vi "Title_Blit.vi"(0 "Title":T2, 5 "Sprites":cluster{"Pix":u8[][], "Mask":u8[][]}[](array[cluster]), 7 "State":T1={"Tick"=0, "Phase"=0, "PhaseTicks"=0, "Level"=1, "Room"=0, "X10"=0, "Y10"=0, "VY10"=0, "Mode"=0, "Facing"=0, "Run"=0, "Vert"=0, "StandY"=0, "EntryX10"=0, "EntryY10"=0, "EntryMode"=0, "Lives"=4, "Score"=0, "NextLife"=10000, "KeyR"=0, "KeyB"=0, "KeyY"=0, "Torch"=FALSE, "FloorPhase"=0, "Dead"=FALSE, "LevelStart"=FALSE, "Quit"=FALSE, "Sound"=0, "Seed"=12345, "DemoStep"=0, "Tiles"=[], "World"=[], "Enemies"=[], "Highscores"=[], "Name"=[0, 0, 0], "Cursor"=0}, 11 "error in":errorcluster) -> (4 "Picture":u8[][](array[numeric]), 15 "error out":errorcluster)   [LabVIEW 2020, in "GH_Render.lvlib"]
doc: "The title screen as one raster (rows x width*3 RGB): title.png holds two pages one below the other - the title image and below it the short help (shown TITLE_HELP ticks after the title card) - with the overlay of the phase on top."
uses:
  GH_Render.lvlib
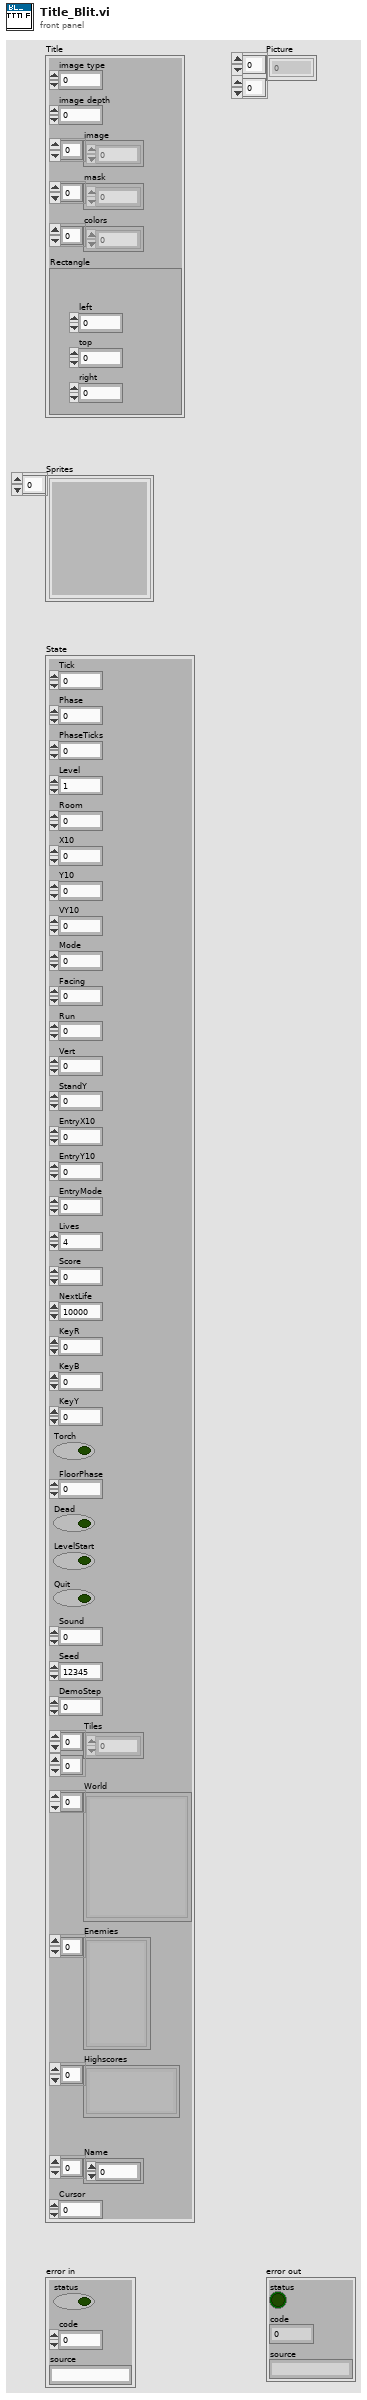
[diagram p1: front panel]
types:
  T1 = cluster{"Tick":u32, "Phase":i32, "PhaseTicks":i32, "Level":i32, "Room":i32, "X10":i32, "Y10":i32, "VY10":i32, "Mode":i32, "Facing":i32, "Run":i32, "Vert":i32, "StandY":i32, "EntryX10":i32, "EntryY10":i32, "EntryMode":i32, "Lives":i32, "Score":i32, "NextLife":i32, "KeyR":i32, "KeyB":i32, "KeyY":i32, "Torch":bool, "FloorPhase":i32, "Dead":bool, "LevelStart":bool, "Quit":bool, "Sound":i32, "Seed":u32, "DemoStep":i32, "Tiles":u8[][], "World":cluster{"ID":string, "Depth":i32, "Column":i32, "Tiles":u8[][]}[], "Enemies":cluster{"Kind":i32, "X10":i32, "Y10":i32, "Dir":i32, "Mode":i32}[], "Highscores":cluster{"Score":i32, "Name":string}[], "Name":i32[], "Cursor":i32}
  T2 = cluster{"image type":i32, "image depth":i32, "image":u8[], "mask":u8[], "colors":u32[], "Rectangle":cluster{"left":i16, "top":i16, "right":i16, "bottom":i16}}
  T3 = cluster{"left":i16, "top":i16, "right":i16, "bottom":i16}
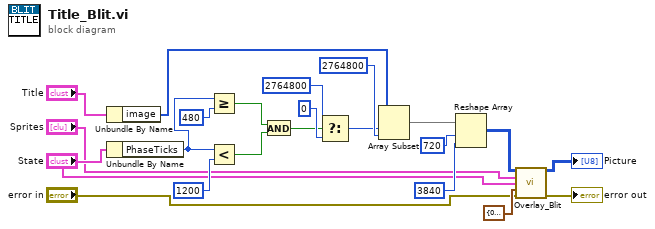
[diagram p0: block diagram]
diagram:
  n1 = Unbundle By Name("Title") -> ("image"=w11:u8[])
  n2 = Unbundle By Name("State") -> ("PhaseTicks"=w5:i32)
  n3 = Greater Or Equal?(x=w5, y=480) -> (x >= y?=w7:bool)
  n4 = Less?(x=w5, y=1200) -> (x < y?=w9:bool)
  n5 = And(x=w7, y=w9) -> (x .and. y?=w10:bool)
  n6 = Select(t=2764800, s=w10, f=0) -> (s? t:f=w14:i32)
  n7 = Array Subset(array=w11, index=w14, length=2764800) -> (w16:u8[])
  n8 = Reshape Array(w16, 720, 3840) -> (w19:u8[][])
  n9 = call "Overlay_Blit.vi"("Picture"=w19, "Sprites"="Sprites", "State"="State", "Clip"=T3 {"left"=0, "top"=0, "right"=1280, "bottom"=720} ("Whole screen"), "error in"="error in") -> ("Picture out"=→"Picture":u8[][], "error out"=→"error out":errorcluster)  [unwired: 9 in]
